vi "VIH - CHM Project - HHP Support - Delete Key.vi"(7 "Section":string, 8 "error in":errorcluster, 10 "Key":string, 11 "queue":T1) -> (0 "error out":errorcluster, 3 "dup queue":T1)   [LabVIEW 2014]
doc: "::: VI Helpeks :::\nCopyright (c) 2000-2026 Konstantin Shifershteyn. All rights reserved."
uses:
  VIH - CHM Project - HHP Support - Queue Refnum.ctl
  VIH - CHM Project - HHP Support - Config Data Cluster.ctl
panel:
  # "VI Helpeks\nCopyright (c) 2012-2026 Konstantin Shifershteyn"
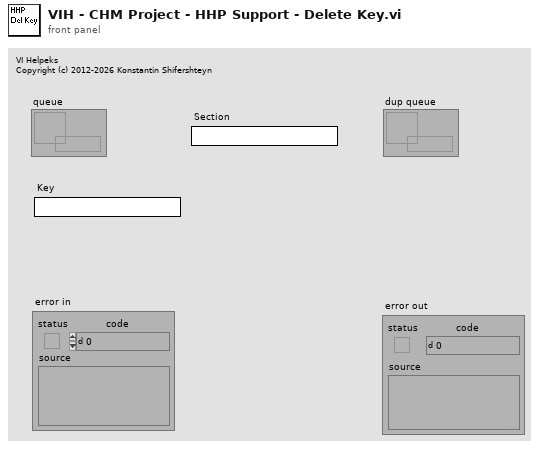
[diagram p1: front panel]
types:
  T1 = typedef "VIH - CHM Project - HHP Support - Queue Refnum.ctl" = refnum<queue>
  T2 = typedef "VIH - CHM Project - HHP Support - Config Data Cluster.ctl" = cluster{"Fille path":path, "sections":cluster{"Sec name":string, "key-values":string[][]}[]}
  T3 = cluster{"Sec name":string, "key-values":string[][]}[]
  T4 = cluster{"Sec name":string, "key-values":string[][]}
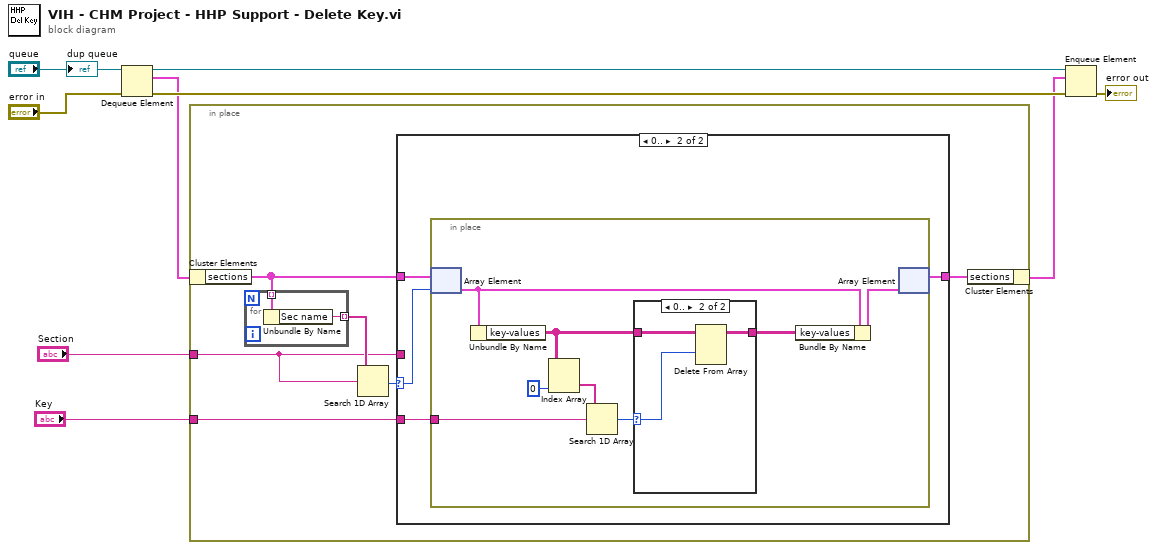
[diagram p0: block diagram]
diagram:
  n1 = Dequeue Element(queue="queue", error in (no error)="error in") -> (queue out=w9:T1, element=w4:T2, error out=w6:errorcluster)  [unwired: 1 in, 1 out]
  n2 = in-place {
    in-place-border: "Section" -> [w11]
    in-place-border: "Key" -> [w10]
    n3 = in-place-cluster #1(w4) -> ("sections"=w13:T3)
    n4 = for {
      tunnel: w13 -> [w34] mode=indexing
      tunnel: [w33] -> w15 mode=indexing
      n5 = Unbundle By Name(w34) -> ("Sec name"=w33:string)
    }
    n6 = Search 1D Array(1D array=w15, element=w11) -> (index of element=w14:i32)  [unwired: 1 in]
    n7 = case shown="0.." w14 {
      selector: w14 -> [_ w18]
      tunnel: w13 -> [w16 w19]
      tunnel: [w16 w17] -> w12
      tunnel: w11 -> [_ _]
      tunnel: w10 -> [_ w20]
      frame ..-1 {
      }
      frame 0.. {
        n8 = in-place {
          in-place-border: w20 -> [w27]
          n9 = in-place-array #2(w19, w18) -> (w24:T4)
          n10 = Unbundle By Name(w24) -> ("key-values"=w22:string[][])
          n11 = Index Array(array=w22, index (col)=0 ("disabled index (col)")) -> (element=w26:string[])  [unwired: 1 in]
          n12 = Search 1D Array(1D array=w26, element=w27) -> (index of element=w25:i32)  [unwired: 1 in]
          n13 = case shown="0.." w25 {
            selector: w25 -> [_ w30]
            tunnel: w22 -> [w29 w32]
            tunnel: [w29 w31] -> w21
            frame ..-1 {
            }
            frame 0.. {
              n14 = Delete From Array(array=w32, index (row)=w30) -> (array with subset deleted=w31:string[][])  [unwired: 2 in, 1 out]
            }
          }
          n15 = Bundle By Name(cluster=w24, "key-values"=w21) -> (w23:T4)
          n16 = in-place-array #2(w23) -> (w17:T3)  [unwired: 1 out]
        }
      }
    }
    n17 = in-place-cluster #1("sections"=w12) -> (w3:T2)
  }
  n18 = Enqueue Element(queue=w9, element=w3, error in (no error)=w6) -> (error out=→"error out":errorcluster)  [unwired: 1 in, 2 out]
  "dup queue" <- "queue"
